vi "GV-SetYstdScale.vi"(8 "error in (no error)":errorcluster, 11 "Gviewer in":refnum<class "Gviewer.lvclass">) -> (0 "error out":errorcluster, 3 "Gviewer out":refnum<class "Gviewer.lvclass">)   [LabVIEW 2020, in "Sgraph_lib_V1.lvlib" / "Gviewer.lvclass"]
doc: "Andre Koelewijn, 30 jan 2021\n\nAdapt the Standard Y scale to one of the TAGs"
uses:
  Gviewer.lvclass
  Gviewer.lvclass/Gviewer.ctl
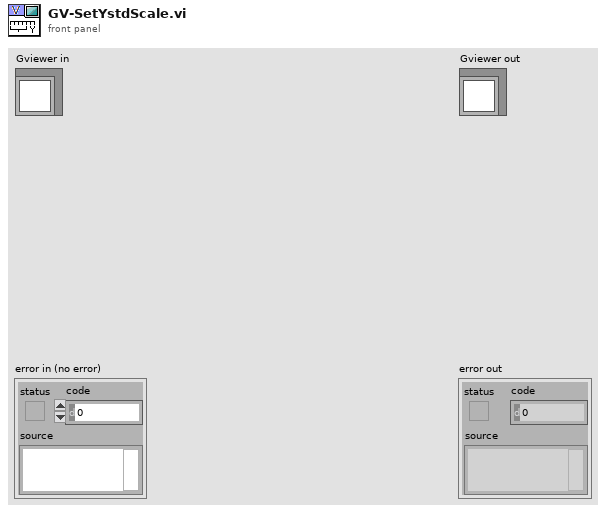
[diagram p1: front panel]
types:
  T1 = typedef "Sgraph_lib_V1.lvlib/Gviewer.lvclass/Typedef_SelProperties.ctl" = cluster{"Color":u32, "LineType":T2, "max":dbl, "min":dbl}
  T2 = typedef "Sgraph_lib_V1.lvlib/Gviewer.lvclass/Typedef_LineType.ctl" = enum16{"num_bare", "num_MinMax_Area", "num_MinMax_Lines", "num_MinMax_Forfor", "num_Max_Area", "num_Max_Line", "num_Max_Forfor", "num_Min_Area", "num_Min_Line", "num_Min_Fosfor", "Boolean_Line_01", "Boolean_Area_01", "Boolean_Fosfor_01", "Boolean_Line_TF", "Boolean_Area_TF", "Boolean_Fosfor_TF", "Boolean_OnOff_Line", "Boolean_OnOff_Area", "Boolean_OnOff_Fosfor", "Boolean_spare", "StringEvent_Line", "StringEvent_TimeLine"}
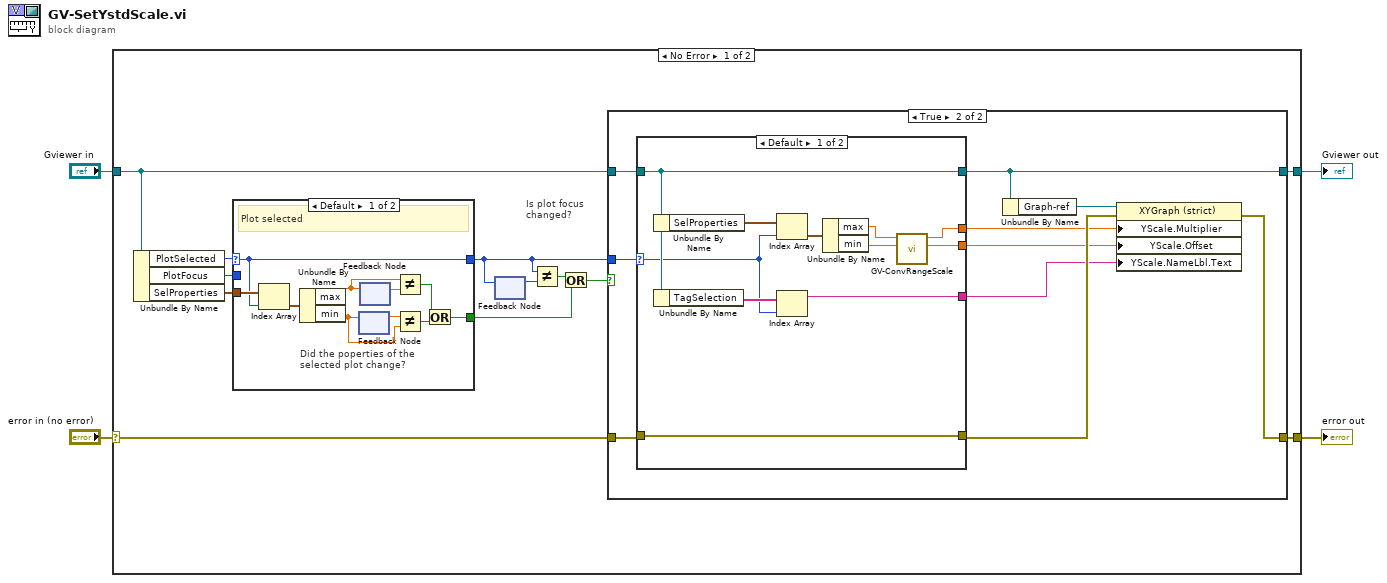
[diagram p0: block diagram]
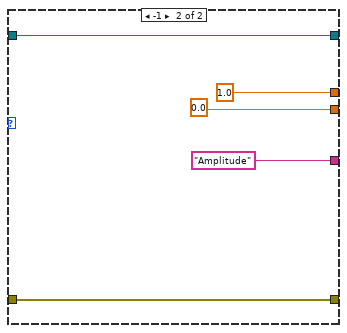
[diagram p3: hidden frame]
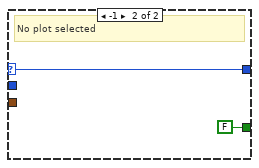
[diagram p4: hidden frame]
diagram:
  n1 = case shown="No Error" "error in (no error)" {
    selector: "error in (no error)" -> [w13 w58]
    tunnel: [w11 w58] -> w3
    tunnel: [w12 w57] -> w1
    tunnel: "Gviewer in" -> [w14 w57]
    frame No Error {
      # "Is plot focus\nchanged?"
      n2 = Unbundle By Name(w14) -> ("PlotSelected"=w16:i32, "PlotFocus"=w15:i32, "SelProperties"=w6:T1[])
      n3 = case shown="Default" w16 {
        selector: w16 -> [w45 w55]
        tunnel: w15 -> [_ _]
        tunnel: [w45 w55] -> w9
        tunnel: w6 -> [w54 _]
        tunnel: [w46 FALSE] -> w5
        frame Default {
          # "Did the poperties of the\nselected plot change?"
          # "Plot selected"
          n4 = Index Array(array=w54, index=w45) -> (element=w53:T1)
          n5 = Unbundle By Name(w53) -> ("max"=w51:dbl, "min"=w49:dbl)
          n6 = feedback #1() -> (w50:dbl)  [unwired: 1 in]
          n7 = feedback-in #1(w49) -> ()
          n8 = feedback #2() -> (w52:dbl)  [unwired: 1 in]
          n9 = feedback-in #2(w51) -> ()
          n10 = Not Equal?(x=w51, y=w52) -> (x != y?=w48:bool)
          n11 = Not Equal?(x=w50, y=w49) -> (x != y?=w47:bool)
          n12 = Or(x=w48, y=w47) -> (x .or. y?=w46:bool)
        }
        frame -1 {
          # "No plot selected"
        }
      }
      n13 = feedback-in #3(w9) -> ()
      n14 = feedback #3() -> (w10:i32)  [unwired: 1 in]
      n15 = Not Equal?(x=w9, y=w10) -> (x != y?=w8:bool)
      n16 = Or(x=w8, y=w5) -> (x .or. y?=w7:bool)
      n17 = case shown="True" w7 {
        tunnel: w9 -> [_ w28]
        tunnel: w14 -> [w17 w27]
        tunnel: w13 -> [w18 w26]
        tunnel: [w17 w24] -> w12
        tunnel: [w18 w22] -> w11
        frame False {
        }
        frame True {
          n18 = case shown="Default" w28 {
            selector: w28 -> [w32 _]
            tunnel: w27 -> [w34 w44]
            tunnel: w26 -> [w39 w43]
            tunnel: [w34 w44] -> w24
            tunnel: [w39 w43] -> w23
            tunnel: [w30 1.0] -> w20
            tunnel: [w29 0.0] -> w19
            tunnel: [w31 "Amplitude" ("Tag")] -> w21
            frame Default {
              n19 = Unbundle By Name(w34) -> ("SelProperties"=w38:T1[])
              n20 = Unbundle By Name(w34) -> ("TagSelection"=w33:string[])
              n21 = Index Array(array=w38, index=w32) -> (element=w37:T1)
              n22 = Index Array(array=w33, index=w32) -> (element=w31:string)
              n23 = Unbundle By Name(w37) -> ("max"=w35:dbl, "min"=w36:dbl)
              n24 = call "GV-ConvRangeScale.vi"("RangeL"=w36, "RangeH"=w35) -> ("Offset"=w29:dbl, "Gain"=w30:dbl)  [unwired: 8 in]
            }
            frame -1 {
            }
          }
          n25 = Unbundle By Name(w24) -> ("Graph-ref"=w25:refnum<vi>)
          n26 = property class="XYGraph (strict)"(reference=w25, error in=w23, "YScale.Multiplier"=w20, "YScale.Offset"=w19, "YScale.NameLbl.Text"=w21) -> (error out=w22:errorcluster)  [unwired: 1 out]
        }
      }
    }
    frame Error {
    }
  }
  "error out" <- w3
  "Gviewer out" <- w1
